vi "FlatToRichcif_can_reader_cansub_Statistics.vi"(5 "OutputClusterType":T1, 11 "InputCluster":T2) -> (3 "OutputCluster":T1)   [LabVIEW 2021, in "CanReaderCansub_server.lvlib"]
uses:
  CanReaderCansub_server.lvlib
  cif_can_reader_cansub_Statistics_Flat.ctl
  cif_can_reader_cansub_Statistics.ctl
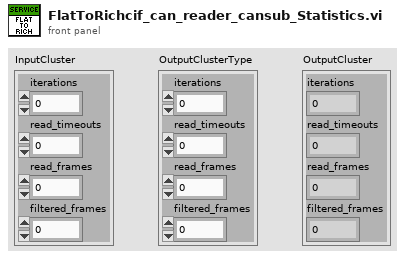
[diagram p1: front panel]
types:
  T1 = typedef "CanReaderCansub_server.lvlib/cif_can_reader_cansub_Statistics.ctl" = cluster{"iterations":u64, "read_timeouts":u64, "read_frames":u64, "filtered_frames":u64}
  T2 = typedef "CanReaderCansub_server.lvlib/cif_can_reader_cansub_Statistics_Flat.ctl" = cluster{"iterations":u64, "read_timeouts":u64, "read_frames":u64, "filtered_frames":u64}
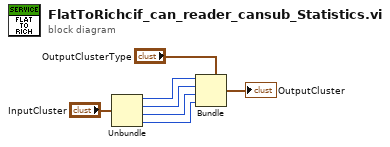
[diagram p0: block diagram]
diagram:
  n1 = Unbundle "Unbundle"("InputCluster") -> ("iterations"=w4:u64, "read_timeouts"=w3:u64, "read_frames"=w2:u64, "filtered_frames"=w1:u64)
  n2 = Bundle "Bundle"(cluster="OutputClusterType", "iterations"=w4, "read_timeouts"=w3, "read_frames"=w2, "filtered_frames"=w1) -> (→"OutputCluster":T1)
